vi "serialization tests.vi"() -> (0 "error out":errorcluster, 1 "modules equal":bool, 2 "lines equal":bool, 3 "channels equal":bool)   [LabVIEW 2015, in "J1939 tests.lvlib"]
doc: "Tests the 'To String' and 'From String' methods of the Module's configuration class and ensures they are compatible."
uses:
  J1939 tests.lvlib
  module/configuration/XNET Settings.ctl
  module/configuration/J1939 configuration.lvclass
  module/configuration/J1939 configuration.lvclass/J1939 configuration.ctl
  module/configuration/Read XNET Settings.vi
  <vilib>/NI/Tag Bus Module Framework/channel/TBM channel.lvclass
panel:
  out "Xnet Settings":bool
  out "XNET Settings 2":T1={"Select Interface"="CAN2", "Claim By Adress"=FALSE, "Node Address"=1, "Node Name"=1}
  out "XNET Settings":T1={"Select Interface"="CAN2", "Claim By Adress"=FALSE, "Node Address"=1, "Node Name"=1}
  out "error in":errorcluster
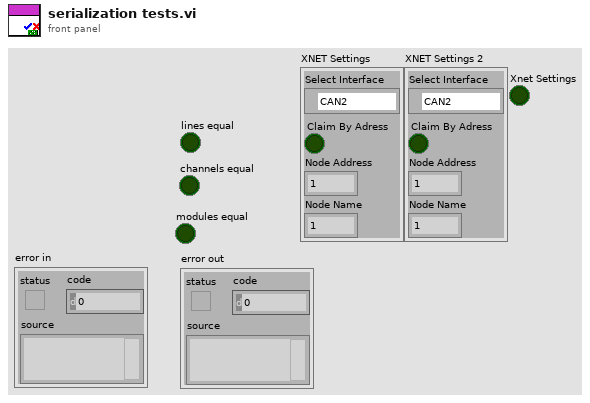
[diagram p1: front panel]
types:
  T1 = typedef "J1939 configuration.lvclass/XNET Settings.ctl" = cluster{"Select Interface":refnum<k21>, "Claim By Adress":bool, "Node Address":u8, "Node Name":u64}
  T2 = typedef "J1939 configuration.lvclass/Line.ctl" = cluster{"channel":refnum<class "TBM channel.lvclass">, "XNET Signal":refnum<k21>}
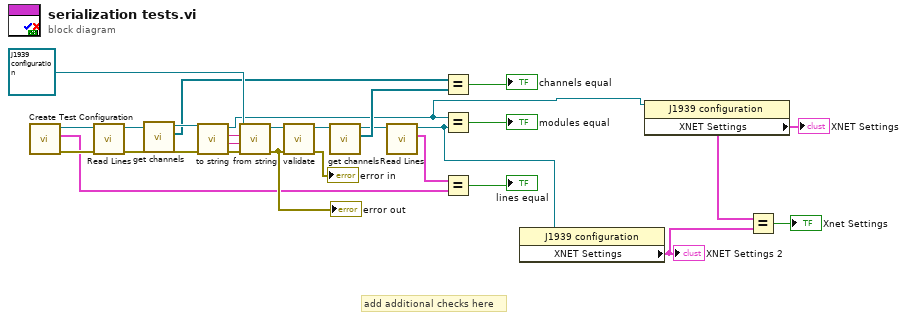
[diagram p0: block diagram]
diagram:
  # "add additional checks here"
  n1 = call "Create Test Configuration.vi"() -> ("error out"=w10:errorcluster, "Line Array"=w6:T2[], "Module Configuration"=w8:refnum<class "J1939 configuration.lvclass">)  [unwired: 5 in, 4 out]
  n2 = call "Read Lines.vi"("error in (no error)"=w10, "J1939 configuration in"=w8) -> ("error out"=w9:errorcluster, "J1939 configuration out"=w7:refnum<class "J1939 configuration.lvclass">)  [unwired: 7 in, 1 out]
  n3 = call-dynamic "get channels.vi"("J1939 configuration in"=w7) -> ("channels"=w14:refnum<class "TBM channel.lvclass">[], "J1939 configuration out"=w15:refnum<class "J1939 configuration.lvclass">)  [unwired: 9 in]
  n4 = call-dynamic "to string.vi"("error in"=w9, "J1939 configuration in"=w15) -> ("error out"=w26:errorcluster, "data"=w25:string, "version"=w24:string, "J1939 configuration out"=w4:refnum<class "J1939 configuration.lvclass">)  [unwired: 6 in]
  n5 = call-dynamic "from string.vi"("error in"=w26, "data"=w25, "version"=w24, "J1939 configuration in"=refnum<class "J1939 configuration.lvclass"> refnum ("tag bus configurable plugin module configuration")) -> ("error out"=w21:errorcluster, "J1939 configuration out"=w23:refnum<class "J1939 configuration.lvclass">)  [unwired: 6 in]
  "error out" <- w21
  n6 = call-dynamic "validate.vi"("error in"=w21, "J1939 configuration in"=w23) -> ("error out"=→"error in":errorcluster, "J1939 configuration out"=w19:refnum<class "J1939 configuration.lvclass">)  [unwired: 8 in]
  n7 = call-dynamic "get channels.vi"("J1939 configuration in"=w19) -> ("channels"=w18:refnum<class "TBM channel.lvclass">[], "J1939 configuration out"=w13:refnum<class "J1939 configuration.lvclass">)  [unwired: 9 in]
  n8 = call "Read Lines.vi"("J1939 configuration in"=w13) -> ("Lines"=w12:T2[], "J1939 configuration out"=w5:refnum<class "J1939 configuration.lvclass">)  [unwired: 8 in, 1 out]
  n9 = Equal?(x=w14, y=w18) -> (x = y?=→"channels equal":bool)
  n10 = Equal?(x=w4, y=w5) -> (x = y?=→"modules equal":bool)
  n11 = Equal?(x=w12, y=w6) -> (x = y?=→"lines equal":bool)
  n12 = property class="J1939 configuration"(reference=w5) -> ("XNET Settings"=w3:T1)  [unwired: 1 in, 2 out]
  "XNET Settings 2" <- w3
  n13 = property class="J1939 configuration"(reference=w4) -> ("XNET Settings"=w2:T1)  [unwired: 1 in, 2 out]
  "XNET Settings" <- w2
  n14 = Equal?(x=w2, y=w3) -> (x = y?=→"Xnet Settings":bool)
